vi "Read String.vi"(8 "error in (no error)":errorcluster, 9 "offset (0)":i64, 10 "bytes to read":i64, 11 "pointer in":u64) -> (0 "error out":errorcluster, 1 "offset out":i64, 2 "string out":string, 3 "pointer out":u64)   [LabVIEW 2016, in "Linux RT IPC.Shared Memory.lvlib"]
uses:
  Linux RT IPC.Shared Memory.lvlib
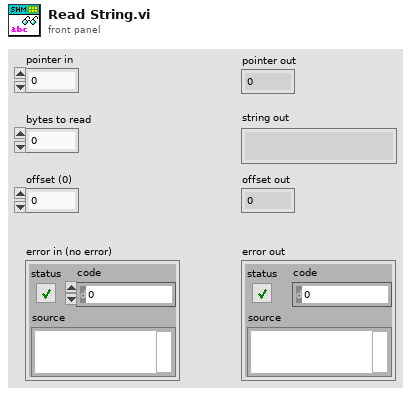
[diagram p1: front panel]
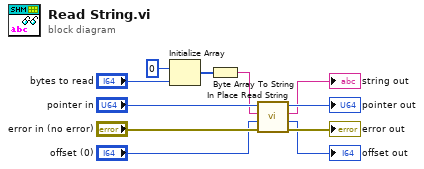
[diagram p0: block diagram]
diagram:
  n1 = Initialize Array(u8 0, "bytes to read") -> (w4:u8[])
  n2 = Byte Array To String(unsigned byte array=w4) -> (string=w3:string)
  n3 = call "In Place Read String.vi"("error in (no error)"="error in (no error)", "offset (0)"="offset (0)", "preallocated string in"=w3, "pointer in"="pointer in") -> ("error out"=→"error out":errorcluster, "offset out"=→"offset out":i64, "string out"=→"string out":string, "pointer out"=→"pointer out":u64)  [unwired: 4 in]
